vi "ClearClassNameCache.vi"(8 "error in (no error)":errorcluster, 11 "ClassName Cache":refnum<data-value>) -> (0 "error out":errorcluster, 3 "ClassName Cache":refnum<data-value>)   [LabVIEW 2020, in "BlueSerialization.lvlib" / "BlueSerializer.lvclass"]
uses:
  BlueSerializer.lvclass
  ClassNameCacheCluster.ctl
  ClassNameCacheMap.ctl
  ClassNameObj.ctl
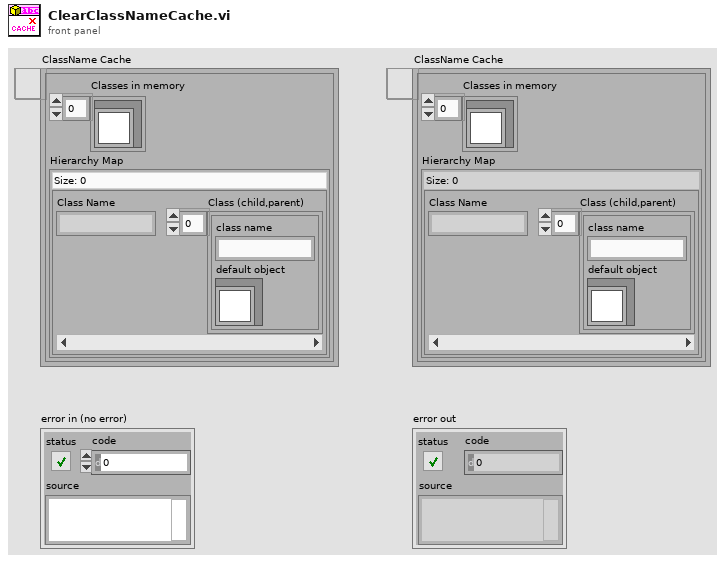
[diagram p1: front panel]
types:
  T1 = typedef "BlueSerialization.lvlib/BlueSerializer.lvclass/ClassNameCacheCluster.ctl" = cluster{"Classes in memory":refnum<class>[], "Hierarchy Map":T2}
  T2 = typedef "BlueSerialization.lvlib/BlueSerializer.lvclass/ClassNameCacheMap.ctl" = map{string, T3[]}
  T3 = typedef "BlueSerialization.lvlib/BlueSerializer.lvclass/ClassNameObj.ctl" = cluster{"class name":string, "default object":refnum<class>}
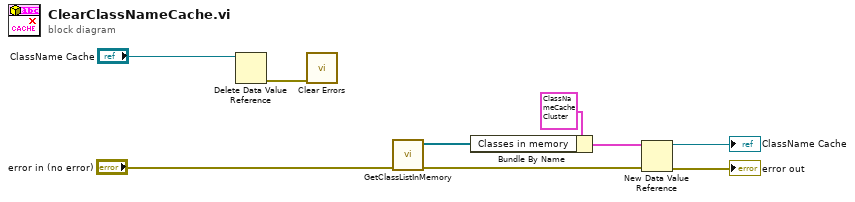
[diagram p0: block diagram]
diagram:
  n1 = Delete Data Value Reference(data value reference="ClassName Cache") -> (error out=w7:errorcluster)  [unwired: 1 in, 1 out]
  n2 = call <vilib>:"Clear Errors.vi"("error in (no error)"=w7) -> ()  [unwired: 5 in, 2 out]
  n3 = call "GetClassListInMemory.vi"("error in (no error)"="error in (no error)") -> ("error out"=w1:errorcluster, "Classes in memory"=w4:refnum<class>[])  [unwired: 9 in]
  n4 = Bundle By Name(cluster=T1 {"Classes in memory"=[], "Hierarchy Map"={}} ("Cluster"), "Classes in memory"=w4) -> (w3:T1)
  n5 = New Data Value Reference(data value=w3, error in=w1) -> (data value reference=→"ClassName Cache":refnum<data-value>, error out=→"error out":errorcluster)
